vi "recursively populate tree ctl.vi"(8 "error in (no error)":errorcluster, 10 "Object path":string="IndivITX/Test1/SA03008N.20190801.000000.itx", 11 "tree ctl ref":refnum<vi>) -> (0 "error out":errorcluster, 3 "reference out":refnum<vi>)   [LabVIEW 2019, in "LV-Data.S3.lvclass"]
uses:
  LV-Data.S3.lvclass
panel:
  in  "Tree":string(tree)
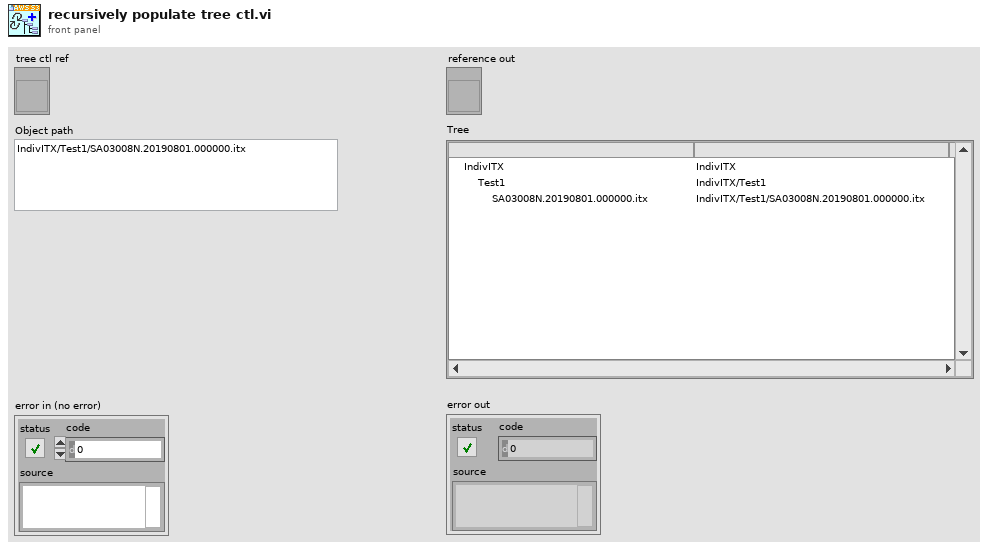
[diagram p1: front panel]
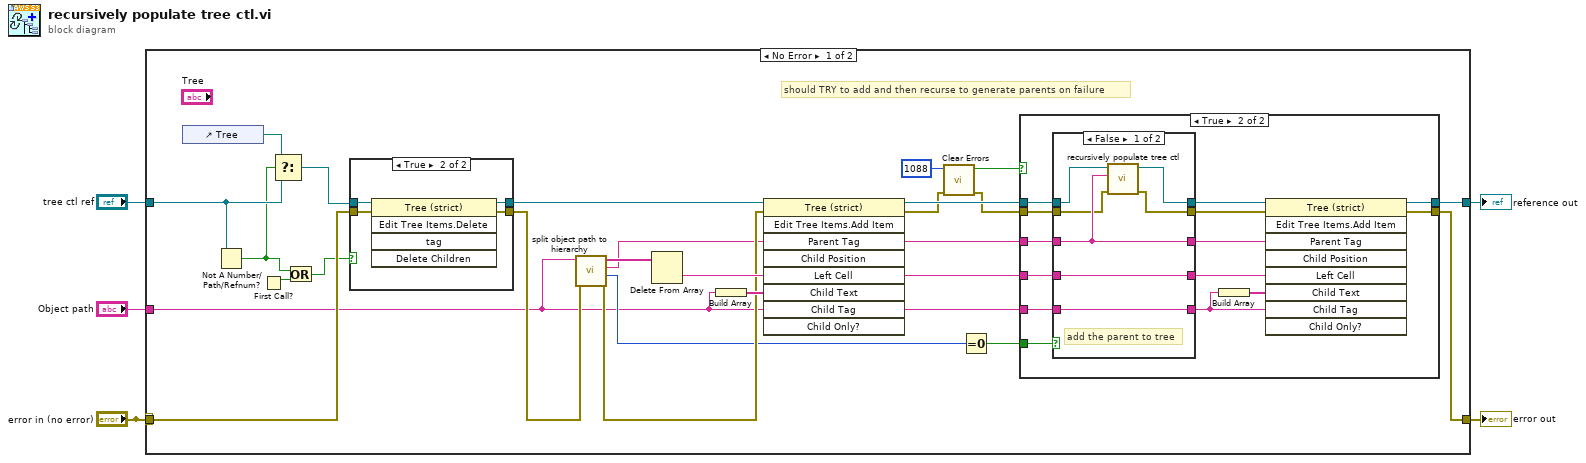
[diagram p0: block diagram]
diagram:
  n1 = case shown="No Error" "error in (no error)" {
    selector: "error in (no error)" -> [_ w64]
    tunnel: [w19 w64] -> w5
    tunnel: [w25 w65] -> w4
    tunnel: "Object path" -> [w10 _]
    tunnel: "tree ctl ref" -> [w9 w65]
    tunnel: "error in (no error)" -> [w12 _]
    frame No Error {
      # "should TRY to add and then recurse to generate parents on failure"
      n2 = control-ref of="Tree"() -> (w20:refnum<vi>)
      n3 = Not A Number/Path/Refnum?(number/path/refnum=w9) -> (NaN/Path/Refnum?=w7:bool)
      n4 = First Call?() -> (First Call?: T/F=w8:bool)
      n5 = Select(t=w20, s=w7, f=w9) -> (s? t:f=w14:refnum<vi>)
      n6 = Or(x=w7, y=w8) -> (x .or. y?=w6:bool)
      n7 = case shown="True" w6 {
        tunnel: w14 -> [w31 w35]
        tunnel: [w31 w34] -> w13
        tunnel: w12 -> [w30 w33]
        tunnel: [w30 w32] -> w11
        frame False {
        }
        frame True {
          n8 = invoke class="Tree (strict)" method="Edit Tree Items.Delete"(reference=w35, error in=w33) -> (reference out=w34:refnum<vi>, error out=w32:errorcluster)  [unwired: 3 in, 3 out]
        }
      }
      n9 = call "split object path to hierarchy.vi"("error in (no error)"=w11, "Object path"=w10) -> ("error out"=w21:errorcluster, "layers"=w16:i32, "parent path"=w15:string, "hierarchy"=w23:string[])  [unwired: 6 in]
      n10 = Delete From Array(array=w23) -> (deleted portion=w22:string)  [unwired: 2 in, 1 out]
      n11 = Build Array(w10) -> (w28:string[])
      n12 = invoke on="Invoke Node" class="Tree (strict)" method="Edit Tree Items.Add Item"(reference=w13, error in=w21, "Parent Tag"=w15, "Left Cell"=w22, "Child Text"=w28, "Child Tag"=w10) -> (reference out=w24:refnum<vi>, error out=w18:errorcluster)  [unwired: 3 in, 7 out]
      n13 = call <vilib>:"Clear Errors.vi"("error in (no error)"=w18, "specific error code to clear (0: all)"=1088) -> ("error out"=w17:errorcluster, "specific error cleared?"=w27:bool)  [unwired: 4 in]
      n14 = Equal To 0?(x=w16) -> (x = 0?=w29:bool)
      n15 = case shown="True" w27 {
        tunnel: [w37 w46] -> w19
        tunnel: w29 -> [_ w51]
        tunnel: [w36 w47] -> w25
        tunnel: w17 -> [w37 w50]
        tunnel: w15 -> [_ w44]
        tunnel: w24 -> [w36 w45]
        tunnel: w10 -> [_ w38]
        tunnel: w22 -> [_ w40]
        frame False {
        }
        frame True {
          n16 = case shown="False" w51 {
            tunnel: w50 -> [w53 w63]
            tunnel: w44 -> [w56 w61]
            tunnel: [w52 w63] -> w49
            tunnel: w45 -> [w57 w62]
            tunnel: [w58 w62] -> w48
            tunnel: [w56 w61] -> w42
            tunnel: [w55 w60] -> w41
            tunnel: w40 -> [w55 w60]
            tunnel: [w54 w59] -> w39
            tunnel: w38 -> [w54 w59]
            frame False {
              # "add the parent to tree"
              n17 = call "recursively populate tree ctl.vi"("error in (no error)"=w53, "Object path"=w56, "tree ctl ref"=w57) -> ("error out"=w52:errorcluster, "reference out"=w58:refnum<vi>)  [unwired: 7 in]
            }
            frame True {
            }
          }
          n18 = Build Array(w39) -> (w43:string[])
          n19 = invoke on="Invoke Node" class="Tree (strict)" method="Edit Tree Items.Add Item"(reference=w48, error in=w49, "Parent Tag"=w42, "Left Cell"=w41, "Child Text"=w43, "Child Tag"=w39) -> (reference out=w47:refnum<vi>, error out=w46:errorcluster)  [unwired: 3 in, 7 out]
        }
      }
    }
    frame Error {
    }
  }
  "error out" <- w5
  "reference out" <- w4
